vi "UI - Initialize IO Variables.vi"(8 "error in (no error)":errorcluster, 11 "Controller Address":string) -> (0 "error out":errorcluster, 3 "IO References":T1)   [LabVIEW 2025]
uses:
  controls/IO References.ctl
panel:
  out "Array 2":errorcluster[](array[cluster])
  out "Array":string[](array[string])
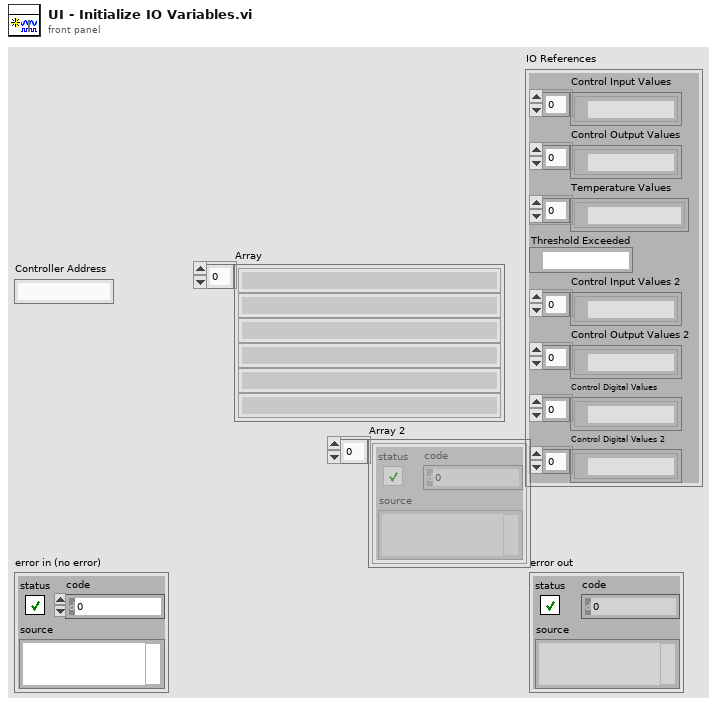
[diagram p1: front panel]
types:
  T1 = typedef "IO References.ctl" = cluster{"Control Input Values":refnum<k21>[], "Control Output Values":refnum<k21>[], "Temperature Values":refnum<k21>[], "Threshold Exceeded":refnum<k21>, "Control Input Values 2":refnum<k21>[], "Control Output Values 2":refnum<k21>[], "Control Digital Values":refnum<k21>[], "Control Digital Values 2":refnum<k21>[]}
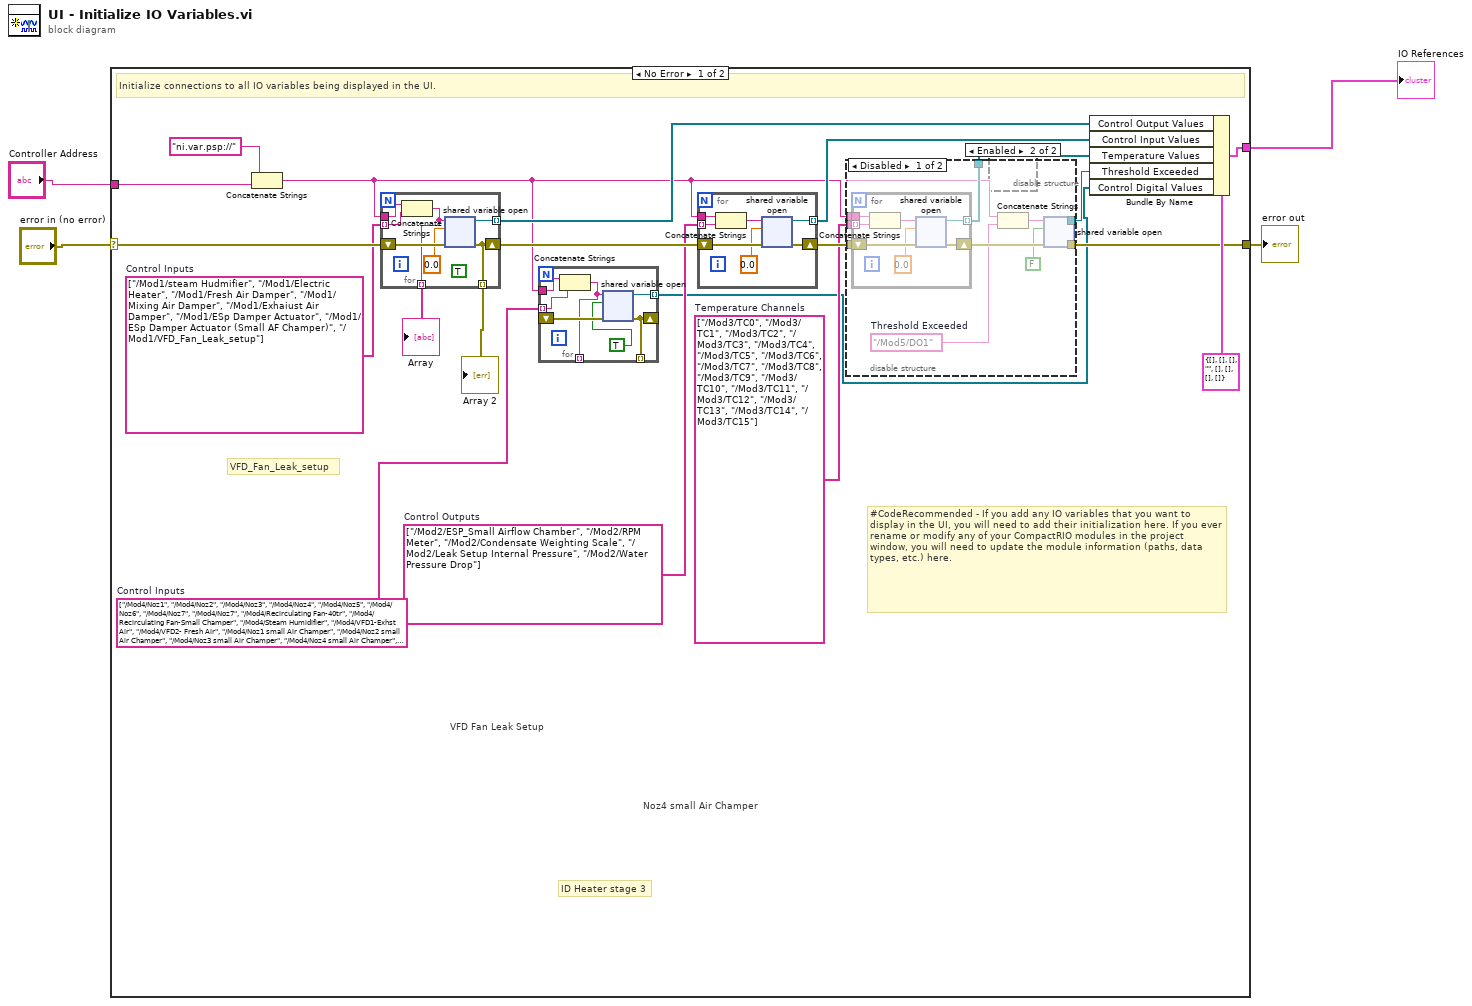
[diagram p0: block diagram]
diagram:
  n1 = case shown="No Error" "error in (no error)" {
    selector: "error in (no error)" -> [w21 w64]
    tunnel: "Controller Address" -> [w23 _]
    tunnel: [w11 w64] -> w2
    tunnel: [w19 _] -> w1
    frame No Error {
      w6 = string[] ["/Mod4/Noz1", "/Mod4/Noz2", "/Mod4/Noz3", "/Mod4/Noz4", "/Mod4/Noz5", "/Mod4/Noz6", "/Mod4/Noz7", "/Mod4/Noz7", "/Mod4/Recirculating Fan-40tr", "/Mod4/Recirculating Fan-Small Champer", "/Mod4/Steam Humidifier", "/Mod4/VFD1-Exhst Air", "/Mod4/VFD2- Fresh Air", "/Mod4/Noz1 small Air Champer", "/Mod4/Noz2 small Air Champer", "/Mod4/Noz3 small Air Champer", "/Mod4/Noz4 small Air Champer", "/Mod4/Noz5 small Air Champer", "/Mod4/VFD Fan Leak Setup", "/Mod4/ID Heater stage 1", "/Mod4/ID Heater stage 2", "/Mod4/ID Heater stage 3", "/Mod4/OD Heater stage 1", "/Mod4/OD Heater stage 2", "/Mod4/OD Heater stage 3", "/Mod4/OD Heater stage 3", "/Mod4/PSY_FAN_Return", "/Mod4/PSY_FAN_Return", "/Mod4/PSY_FAN_Supply", "/Mod4/PSY_FAN_Supply", "/Mod4/PSY_FAN_Ambitient_R", "/Mod4/PSY_FAN_Ambitient_L", "/Mod4/PSY_FAN_AF", "/Mod4/AUX Chiller Pump_1", "/Mod4/AUX Chiller Pump_2"]  # Control Inputs
      w14 = string[] ["/Mod3/TC0", "/Mod3/TC1", "/Mod3/TC2", "/Mod3/TC3", "/Mod3/TC4", "/Mod3/TC5", "/Mod3/TC6", "/Mod3/TC7", "/Mod3/TC8", "/Mod3/TC9", "/Mod3/TC10", "/Mod3/TC11", "/Mod3/TC12", "/Mod3/TC13", "/Mod3/TC14", "/Mod3/TC15"]  # Temperature Channels
      w17 = string[] ["/Mod2/ESP_Small Airflow Chamber", "/Mod2/RPM Meter", "/Mod2/Condensate Weighting Scale", "/Mod2/Leak Setup Internal Pressure", "/Mod2/Water Pressure Drop"]  # Control Outputs
      w20 = string[] ["/Mod1/steam Hudmifier", "/Mod1/Electric Heater", "/Mod1/Fresh Air Damper", "/Mod1/Mixing Air Damper", "/Mod1/Exhaiust Air Damper", "/Mod1/ESp Damper Actuator", "/Mod1/ESp Damper Actuator (Small AF Champer)", "/Mod1/VFD_Fan_Leak_setup"]  # Control Inputs
      # "VFD_Fan_Leak_setup"
      # "ID Heater stage 3"
      # "VFD Fan Leak Setup"
      # "Noz4 small Air Champer"
      # "#CodeRecommended - If you add any IO variables that you want to display in the UI, you will need to add their initialization here. If you ever rename or modify any of your CompactRIO modules in the project window, you will need to update the module information (paths, data types, etc.) here."
      # "Initialize connections to all IO variables being displayed in the UI."
      n2 = Concatenate Strings("ni.var.psp://", w23) -> (w7:string)
      n3 = for {
        shift-right: [w58] -> w18
        shift-left: w21 -> [w63]
        tunnel: w7 -> [w62]
        tunnel: w20 -> [w60] mode=indexing
        tunnel: [w61] -> w8 mode=indexing
        tunnel: [w59] -> w10 mode=indexing
        tunnel: [w58] -> w9 mode=indexing
        (unwired) TRUE
        n4 = Concatenate Strings(w62, w60) -> (w59:string)
        n5 = shared-variable-open(w59, w63, 0.0) -> (w61:refnum<k21>, w58:errorcluster)  [unwired: 1 in]
      }
      "Array" <- w10
      "Array 2" <- w9
      n6 = for {
        shift-right: [w27] -> _
        shift-left: _ -> [w31]
        tunnel: w7 -> [w30]
        tunnel: [w29] -> w5 mode=indexing
        tunnel: [w28] -> _ mode=indexing
        tunnel: [w27] -> _ mode=indexing
        tunnel: w6 -> [w26] mode=indexing
        n7 = Concatenate Strings(w30, w26) -> (w28:string)
        n8 = shared-variable-open(w28, w31, TRUE) -> (w29:refnum<k21>, w27:errorcluster)  [unwired: 1 in]
      }
      n9 = for {
        shift-right: [w55] -> w15
        shift-left: w18 -> [w56]
        tunnel: w7 -> [w52]
        tunnel: w17 -> [w51] mode=indexing
        tunnel: [w50] -> w16 mode=indexing
        n10 = Concatenate Strings(w52, w51) -> (w54:string)
        n11 = shared-variable-open(w54, w56, 0.0) -> (w50:refnum<k21>, w55:errorcluster)  [unwired: 1 in]
      }
      n12 = disable-structure shown="Disabled" {
        disable-tunnel: w15 -> [w41 w49]
        disable-tunnel: w14 -> [w40 _]
        disable-tunnel: [w39 _] -> w13
        disable-tunnel: w7 -> [w38 _]
        disable-tunnel: [w33 _] -> w12
        disable-tunnel: [w32 w49] -> w11
        frame Disabled {
          w36 = "/Mod5/DO1"  # Threshold Exceeded
          n13 = for {
            shift-right: [w47] -> w37
            shift-left: w41 -> [w48]
            tunnel: w38 -> [w44]
            tunnel: w40 -> [w43] mode=indexing
            tunnel: [w42] -> w39 mode=indexing
            n14 = Concatenate Strings(w44, w43) -> (w46:string)
            n15 = shared-variable-open(w46, w48, 0.0) -> (w42:refnum<k21>, w47:errorcluster)  [unwired: 1 in]
          }
          n16 = Concatenate Strings(w38, w36) -> (w35:string)
          n17 = shared-variable-open(w35, w37, FALSE) -> (w33:refnum<k21>, w32:errorcluster)  [unwired: 1 in]
        }
        frame Enabled {
        }
      }
      n18 = disable-structure shown="Enabled" {
        frame Disabled {
        }
        frame Enabled {
        }
      }
      n19 = Bundle By Name(cluster=T1 {"Control Input Values"=[], "Control Output Values"=[], "Temperature Values"=[], "Threshold Exceeded"="", "Control Input Values 2"=[], "Control Output Values 2"=[], "Control Digital Values"=[], "Control Digital Values 2"=[]} ("IO References"), "Control Output Values"=w8, "Control Input Values"=w16, "Temperature Values"=w13, "Threshold Exceeded"=w12, "Control Digital Values"=w5) -> (w19:T1)
    }
    frame Error {
      # "Error"
    }
  }
  "error out" <- w2
  "IO References" <- w1
